vi "csb decode ws to can.vi"(0 "ws_state":u8[](array[numeric]), 1 "hdlc_state":u8[](array[numeric]), 2 "id":u32[](array[numeric]), 3 "dlc":u8[](array[numeric]), 4 "in":u8[](array[numeric]), 5 "ping_payload":u8[](array[numeric]), 6 "t_dev":dbl[](array[numeric]), 7 "error in (no error)":errorcluster, 8 "data":u8[](array[numeric]), 9 "flags":u16[](array[numeric]), 11 "data_len":u8[](array[numeric])) -> (10 "function return":i32, 12 "crc_errors":u32, 14 "decode_errors":i32, 15 "ping_len":i32, 16 "dlc out":u8[](array[numeric]), 17 "data_len out":u8[](array[numeric]), 18 "id out":u32[](array[numeric]), 19 "flags out":u16[](array[numeric]), 20 "ws_state out":u8[](array[numeric]), 21 "data out":u8[](array[numeric]), 22 "hdlc_state out":u8[](array[numeric]), 23 "n_frames":i32, 24 "peer_close":i32, 25 "ping_payload out":u8[](array[numeric]), 26 "t_dev out":dbl[](array[numeric]), 27 "error out":errorcluster)   [LabVIEW 2021, in "CANsub_Codec.lvlib"]
doc: "int32_t csb_decode_ws_to_can(uint8_t *ws_state, int32_t ws_state_size,\n uint8_t *hdlc_state, int32_t hdlc_state_size,\n const uint8_t *in, int32_t in_len,\n double *t_dev, uint32_t *id, uint16_t *flags, uint8_t *dlc,\n uint8_t *data_len, uint8_t *data, int32_t max_frames,\n int32_t *n_frames, int32_t *peer_close,\n uint8_t *ping_payload, int32_t *ping_len,\n uint32_t *crc_errors, int32_t *decode_errors);"
uses:
  CANsub_Codec.lvlib
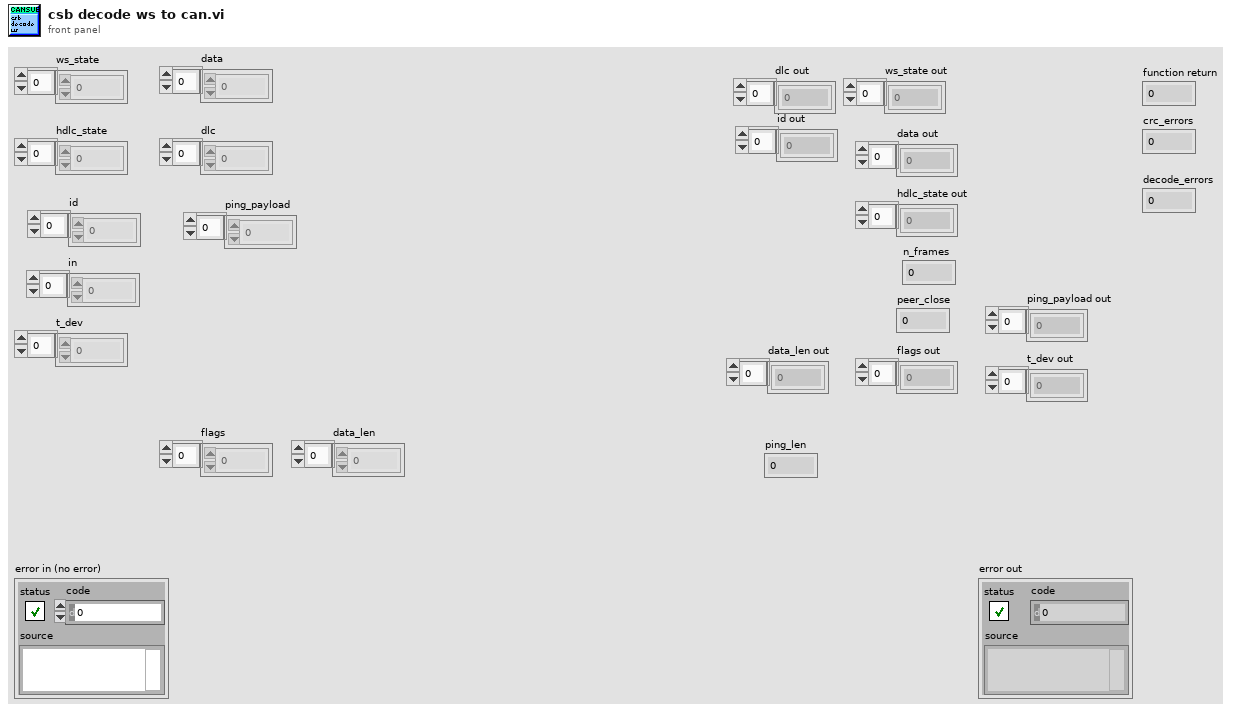
[diagram p1: front panel]
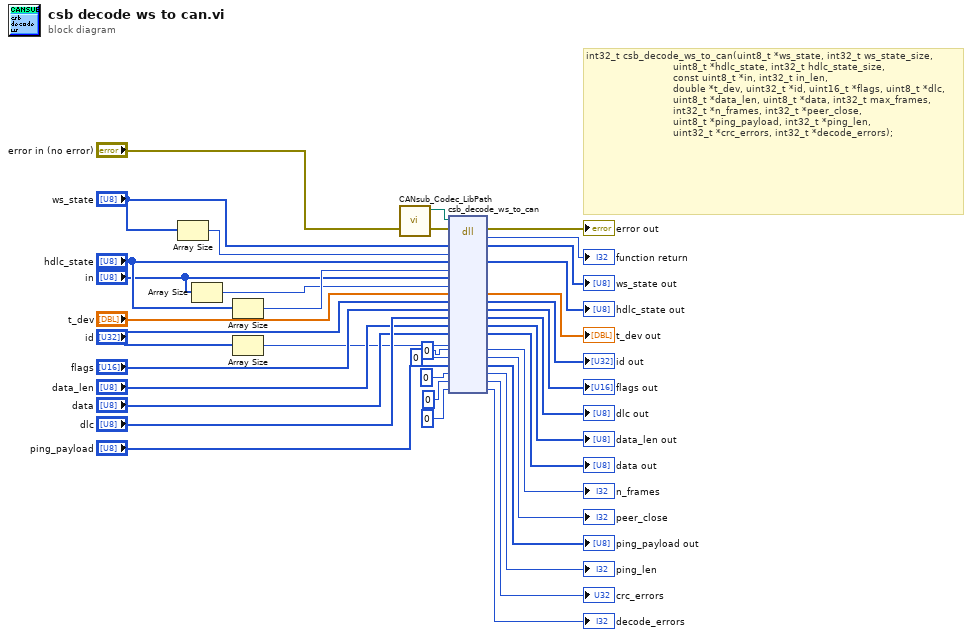
[diagram p0: block diagram]
diagram:
  # "int32_t csb_decode_ws_to_can(uint8_t *ws_state, int32_t ws_state_size,\n                             uint8_t *hdlc_state, int32_t hdlc_state_size,\n                             const uint8_t *in, int32_t in_len,\n                             double *t_dev, uint32_t *id, uint16_t *flags, uint8_t *dlc,\n                             uint8_t *data_len, uint8_t *data, int32_t max_frames,\n                             int32_t *n_frames, int32_t *peer_close,\n                             uint8_t *ping_payload, int32_t *ping_len,\n                             uint32_t *crc_errors, int32_t *decode_errors);"
  n1 = Array Size(array="ws_state") -> (size(s)=w7:i32)
  n2 = Array Size(array="in") -> (size(s)=w3:i32)
  n3 = Array Size(array="hdlc_state") -> (size(s)=w5:i32)
  n4 = Array Size(array="id") -> (size(s)=w1:i32)
  n5 = call "CANsub_Codec_LibPath.vi"() -> ("Path"=w9:path)  [unwired: 11 in]
  n6 = dll-call lib="libcansub_codec.*" fn="csb_decode_ws_to_can"(path in=w9, error in="error in (no error)", "ws_state"="ws_state", "ws_state_size"=w7, "hdlc_state"="hdlc_state", "hdlc_state_size"=w5, "in"="in", "in_len"=w3, "t_dev"="t_dev", "id"="id", "flags"="flags", "dlc"="dlc", "data_len"="data_len", "data"="data", "max_frames"=w1, "n_frames"=0, "peer_close"=0, "ping_payload"="ping_payload", "ping_len"=0, "crc_errors"=u32 0, "decode_errors"=0) -> (error out=→"error out":errorcluster, "return type"=→"function return":i32, "ws_state"=→"ws_state out":u8[], "hdlc_state"=→"hdlc_state out":u8[], "t_dev"=→"t_dev out":dbl[], "id"=→"id out":u32[], "flags"=→"flags out":u16[], "dlc"=→"dlc out":u8[], "data_len"=→"data_len out":u8[], "data"=→"data out":u8[], "n_frames"=→"n_frames":i32, "peer_close"=→"peer_close":i32, "ping_payload"=→"ping_payload out":u8[], "ping_len"=→"ping_len":i32, "crc_errors"=→"crc_errors":u32, "decode_errors"=→"decode_errors":i32)  [unwired: 6 in, 1 out]
